vi "VIH ProjFile - File Tree - Read.vi"(4 "Tree Parent Tag":string, 6 "Project Tree":T1, 8 "error in":errorcluster, 10 "Project Folder":path, 11 "XML Parent Item":refnum<k20>) -> (0 "error out":errorcluster, 3 "dup XML Parent Item":refnum<k20>)   [LabVIEW 2014]
doc: "::: VI Helpeks :::\nCopyright (c) 2000-2026 Konstantin Shifershteyn. All rights reserved."
uses:
  _VIH Project Manager.llb/VIH Project Tree Typedef - Tree Refnum.ctl
  <vilib>/xml/Close Reference(Node).vi
  <vilib>/xml/Close Reference(NNMap).vi
  <resource>/objmgr/DOMUserDefRef.rc
  <vilib>/xml/NI_XML.lvlib
panel:
  # "VI Helpeks\nCopyright (c) 2012-2026 Konstantin Shifershteyn"
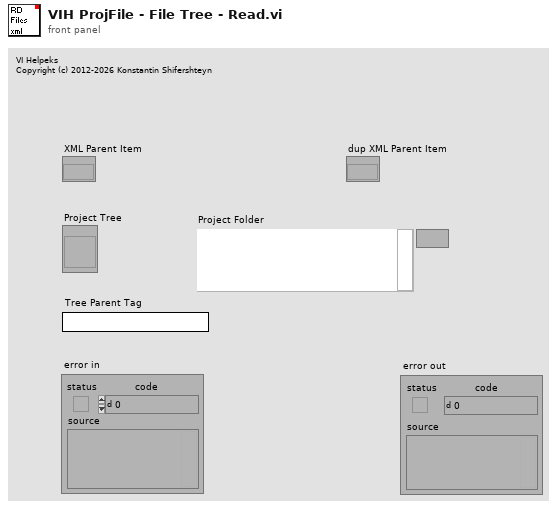
[diagram p1: front panel]
types:
  T1 = typedef "VIH Project Tree Typedef - Tree Refnum.ctl" = refnum<vi>
  T2 = enum16{"get", "get all", "set", "Init", "delete"}
  T3 = typedef "VIH HelpGen Typedef - Cluster - Group Rule.ctl" = cluster{"Source Root Dir":path, "Build Root Dir":path, "BuildHelp":T4, "Source Paths":T5, "Target Paths":T6, "VIDscrMode":T7, "MenuDscrMode":T7, "MenuItemIcons":T4, "Control Rules":T8[], "Flags":T10, "Ctl_DscrMode":T7, "Ctl_ClustMembers":T4, "Ctl_EnumValues":T4, "%Comments":string, "PVIIDscrMode":T7, "VIDetailsMode":T7, "ProductInfoMode":T4, "ProductInfoText":string}
  T4 = typedef "VIH HelpGen Typedef - Enum - Default,Enable,Disable.ctl" = enum16{"Default", "Enable", "Disable"}
  T5 = typedef "VIH HelpGen Typedef - Cluster - Group Rule - Source Paths.ctl" = cluster{"CSS Files":path[], "JS Files":path[], "VI Template":path, "Menu Template":path, "PolyVI Template":path}
  T6 = typedef "VIH HelpGen Typedef - Cluster - Group Rule - Target Paths.ctl" = cluster{"HTML Dir":path, "Image Dir":path, "CSS Dir":path, "JS Dir":path}
  T7 = typedef "VIH HelpGen Typedef - Enum - Description Mode.ctl" = enum16{"Default", "Description", "Description1", "Description2", "Custom", "None"}
  T8 = typedef "VIH HelpGen Typedef - Cluster - Control Rule.ctl" = cluster{"CtrlID":string, "CustomRule":bool, "DscrMode":T7, "Description":string, "ClusterMembers":T4, "EnumValues":T4, "EnumValDscr":T9[], "CustomName":string}
  T9 = typedef "VIH HelpGen Typedef - Cluster - Enum Value Info.ctl" = cluster{"Value":ext, "String":string, "Description":string}
  T10 = typedef "VIH HelpGen Typedef - Cluster - Group Rule - Flags.ctl" = cluster{"Override CSS Files":bool, "Override JS Files":bool, "Override Ctl Rules":bool}
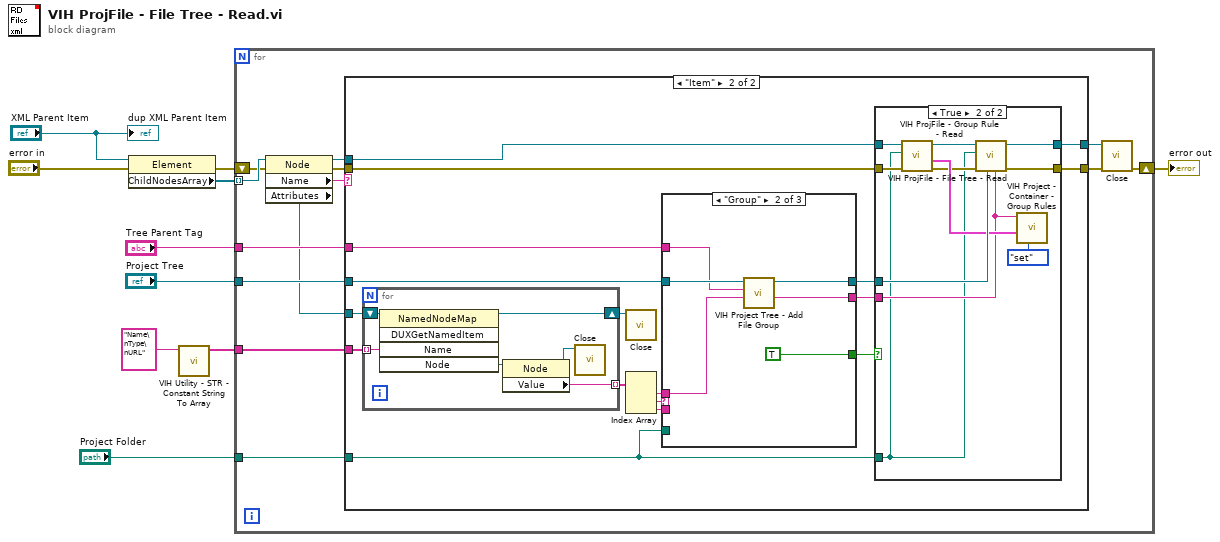
[diagram p0: block diagram]
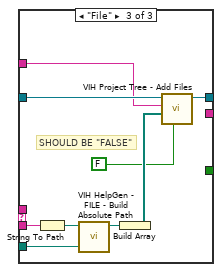
[diagram p4: hidden frame]
diagram:
  n1 = property class="Element"(reference="XML Parent Item", error in="error in") -> (error out=w5:errorcluster, "ChildNodesArray"=w6:refnum<k20>[])  [unwired: 1 out]
  n2 = call "VIH Utility - STR - Constant String To Array.vi"("String in"="Name\nType\nURL") -> ("Array out"=w2:string[])  [unwired: 10 in]
  n3 = for {
    shift-right: [w23] -> w10
    shift-left: w5 -> [w17]
    tunnel: w6 -> [w18] mode=indexing
    tunnel: "Project Tree" -> [w20]
    tunnel: "Tree Parent Tag" -> [w19]
    tunnel: w2 -> [w12]
    tunnel: "Project Folder" -> [w11]
    n4 = property class="Node"(reference=w18, error in=w17) -> (reference out=w14:refnum<k20>, error out=w15:errorcluster, "Name"=w16:string, "Attributes"=w13:refnum<k20>)
    n5 = case shown="\"Item\"" w16 {
      tunnel: [w25 w42] -> w22
      tunnel: [w24 w41] -> w21
      tunnel: w20 -> [_ w40]
      tunnel: w19 -> [_ w39]
      tunnel: w15 -> [w25 w28]
      tunnel: w14 -> [w24 w30]
      tunnel: w13 -> [_ w35]
      tunnel: w12 -> [_ w34]
      tunnel: w11 -> [_ w26]
      frame Default {
      }
      frame "Item" {
        n6 = for {
          tunnel: w34 -> [w61] mode=indexing
          tunnel: [w60] -> w36 mode=indexing
          shift-right: [w59] -> w27
          shift-left: w35 -> [w64]
          n7 = invoke class="NamedNodeMap" method="DUXGetNamedItem"(reference=w64, "Name"=w61) -> (reference out=w59:refnum<k20>, "Node"=w63:refnum<k20>)  [unwired: 3 in, 3 out]
          n8 = property class="Node"(reference=w63) -> (reference out=w62:refnum<k20>, "Value"=w60:string)  [unwired: 1 in, 1 out]
          n9 = call-poly <vilib>:"Close.vi"("node"=w62) -> ()  [unwired: 8 in, 1 out]
        }
        n10 = call-poly <vilib>:"Close.vi"("named node map"=w27) -> ()  [unwired: 8 in, 1 out]
        n11 = Index Array(array=w36) -> (element #1=w33:string, element #2=w32:string, element #3=w29:string)  [unwired: 3 in]
        n12 = case shown="\"Group\"" w32 {
          tunnel: w40 -> [w43 w48 w58]
          tunnel: w39 -> [_ w47 w56]
          tunnel: [_ w44 _] -> w38
          tunnel: [w43 w45 w57] -> w37
          tunnel: w33 -> [_ w46 _]
          tunnel: [_ TRUE _] -> w31
          tunnel: w29 -> [_ _ w54]
          tunnel: w26 -> [_ _ w51]
          frame Default {
          }
          frame "Group" {
            n13 = call "VIH Project Tree - Add File Group.vi"("Group Name"=w46, "Tree Parent Tag"=w47, "Project Tree"=w48) -> ("Item Tag"=w44:string, "dup Project Tree"=w45:T1)  [unwired: 5 in, 2 out]
          }
          frame "File" {
            # "SHOULD BE \"FALSE\""
            n14 = String To Path(string=w54) -> (path=w53:path)
            n15 = call "VIH HelpGen - FILE - Build Absolute Path.vi"("Root Path"=w51, "Path in"=w53) -> ("Path out"=w52:path)  [unwired: 9 in]
            n16 = Build Array(w52) -> (w55:path[])
            n17 = call "VIH Project Tree - Add Files.vi"("Ena dialog message (F)"=FALSE, "File Paths"=w55, "Tree Parent Tag"=w56, "Project Tree"=w58) -> ("dup Project Tree"=w57:T1)  [unwired: 4 in, 3 out]
          }
        }
        n18 = case shown="True" w31 {
          tunnel: w28 -> [w66 w72]
          tunnel: w30 -> [w65 w70]
          tunnel: w37 -> [_ w77]
          tunnel: [w66 w76] -> w42
          tunnel: [w65 w68] -> w41
          tunnel: w38 -> [_ w73]
          tunnel: w26 -> [_ w67]
          frame False {
          }
          frame True {
            n19 = call "VIH ProjFile - Group Rule - Read.vi"("error in"=w72, "Project Folder"=w67, "XML Parent Item"=w70) -> ("error out"=w71:errorcluster, "Group Rule out"=w74:T3, "dup XML Parent Item"=w69:refnum<k20>)  [unwired: 5 in, 1 out]
            n20 = call "VIH ProjFile - File Tree - Read.vi"("Tree Parent Tag"=w73, "Project Tree"=w77, "error in"=w71, "Project Folder"=w67, "XML Parent Item"=w69) -> ("error out"=w76:errorcluster, "dup XML Parent Item"=w68:refnum<k20>)  [unwired: 5 in]
            n21 = call "VIH Project - Container - Group Rules.vi"("cmd (get)"=T2."set", "Group Rule"=w74, "Group ID"=w73) -> ()  [unwired: 4 in, 5 out]
          }
        }
      }
    }
    n22 = call-poly <vilib>:"Close.vi"("error in (no error)"=w22, "node"=w21) -> ("error out"=w23:errorcluster)  [unwired: 7 in]
  }
  "error out" <- w10
  "dup XML Parent Item" <- "XML Parent Item"
